vi "from string.vi"(8 "error in":errorcluster, 9 "data":string, 10 "version":string, 11 "J1939 configuration in":refnum<class "J1939 configuration.lvclass">) -> (0 "error out":errorcluster, 3 "J1939 configuration out":refnum<class "J1939 configuration.lvclass">)   [LabVIEW 2015, in "J1939 configuration.lvclass"]
doc: "Provides an interface for loading a module configuration from a file or other serialized data source. It is recommended that all children of this class store data in two sets--data required for its own initialization, and any data required for parent initialization--and that each implementation uses the <b>Call Parent Method</b> primitive to de-serialize parent information. As a result, it is expected that every module configuration class calls <b>component configuration.lvclass:From String.vi</b>."
uses:
  J1939 configuration.lvclass
  XNET Settings.ctl
  <vilib>/NI/Tag Bus Module Framework/channel/TBM channel.lvclass
  Line.ctl
  J1939 configuration.lvclass/J1939 configuration.ctl
  <vilib>/NI/Tag Bus Module Framework/module configuration/TBM module configuration.lvclass
  <vilib>/NI/Configuration Framework/serializable configuration/NISE_CEF_serializable configuration.lvclass
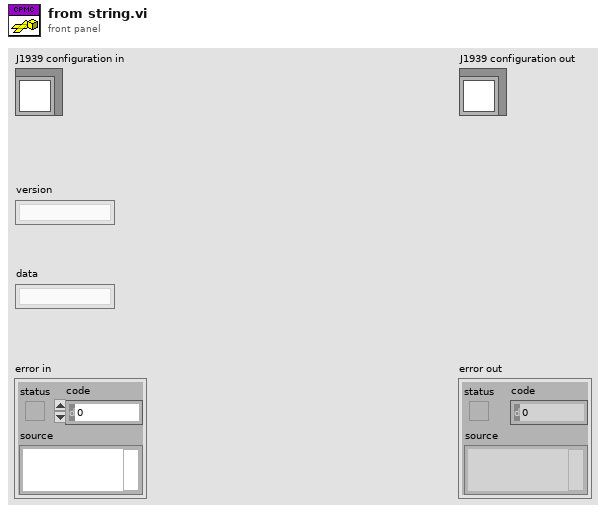
[diagram p1: front panel]
types:
  T1 = typedef "J1939 configuration.lvclass/XNET Settings.ctl" = cluster{"Select Interface":refnum<k21>, "Claim By Adress":bool, "Node Address":u8, "Node Name":u64}
  T2 = typedef "J1939 configuration.lvclass/Line.ctl" = cluster{"channel":refnum<class "TBM channel.lvclass">, "XNET Signal":refnum<k21>}
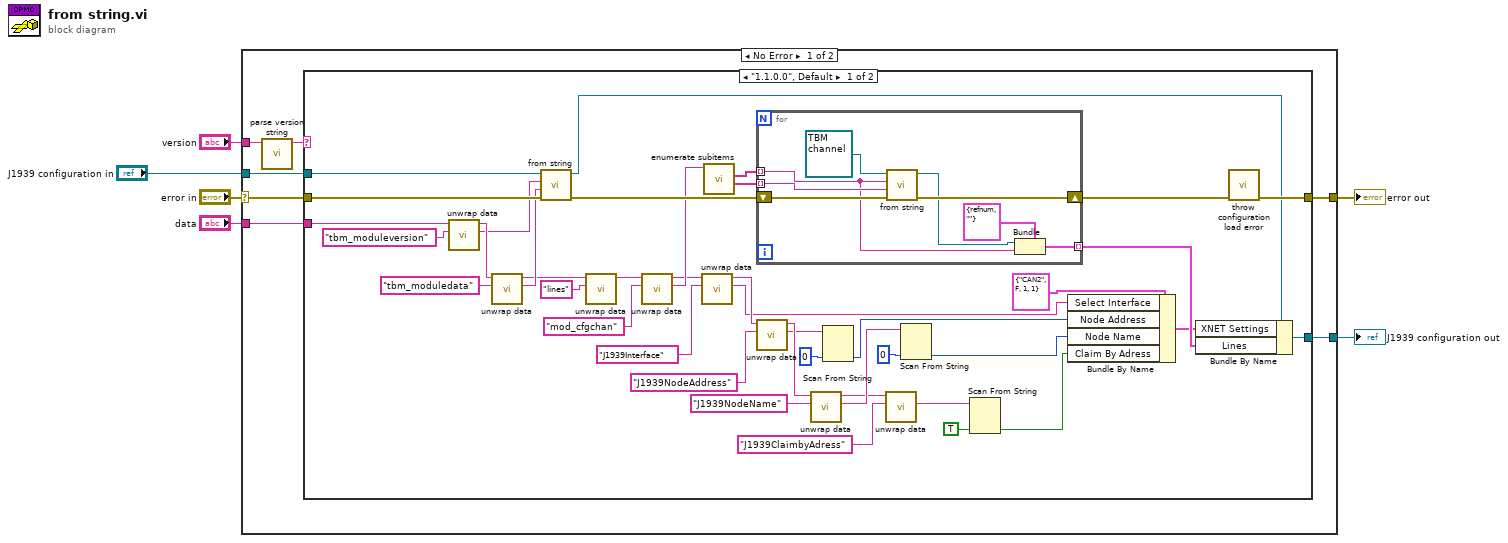
[diagram p0: block diagram]
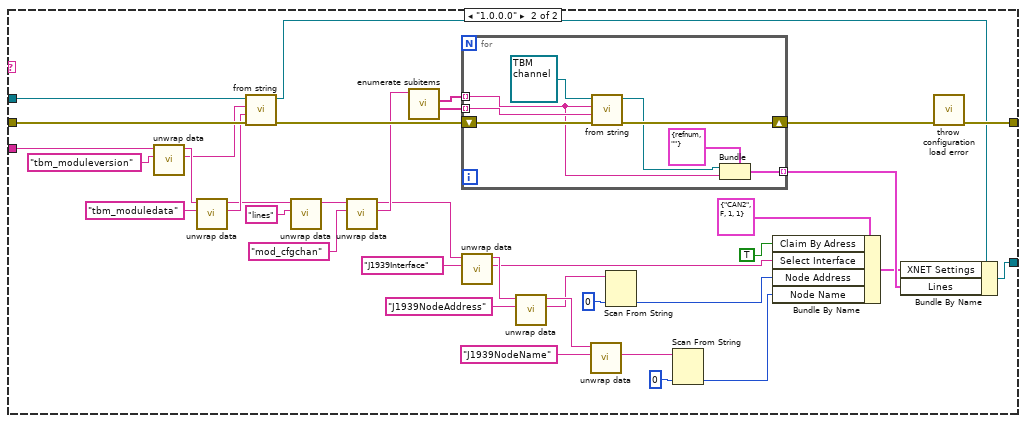
[diagram p2: hidden frame]
diagram:
  n1 = case shown="No Error" "error in" {
    selector: "error in" -> [w7 w109]
    tunnel: "data" -> [w13 _]
    tunnel: "J1939 configuration in" -> [w12 w108]
    tunnel: [w11 w108] -> w5
    tunnel: [w10 w109] -> w4
    tunnel: "version" -> [w9 _]
    frame No Error {
      n2 = call <vilib>:"parse version string.vi"("full version"=w9) -> ("major.minor version"=w8:string)  [unwired: 7 in, 3 out]
      n3 = case shown="\"1.1.0.0\", Default" w8 {
        tunnel: w13 -> [w51 w96]
        tunnel: w7 -> [w50 w95]
        tunnel: w12 -> [w54 w99]
        tunnel: [w42 w87] -> w11
        tunnel: [w53 w98] -> w10
        frame "1.1.0.0", Default {
          n4 = call <vilib>:"unwrap data.vi"("identifier"="tbm_moduleversion" ("additional identifier"), "data to unwrap"=w51) -> ("unwrapped data"=w46:string, "remaining string"=w52:string)  [unwired: 8 in]
          n5 = call <vilib>:"unwrap data.vi"("identifier"="tbm_moduledata" ("additional identifier"), "data to unwrap"=w52) -> ("unwrapped data"=w48:string, "remaining string"=w45:string)  [unwired: 8 in]
          n6 = call-parent "from string.vi"("error in"=w50, "data"=w48, "version"=w46, "module configuration in"=w54) -> ("error out"=w37:errorcluster, "module configuration out"=w43:refnum<class "J1939 configuration.lvclass">)  [unwired: 6 in]
          n7 = call <vilib>:"unwrap data.vi"("identifier"="lines" ("additional identifier"), "data to unwrap"=w45) -> ("remaining string"=w41:string)  [unwired: 8 in, 1 out]
          n8 = call <vilib>:"unwrap data.vi"("identifier"="mod_cfgchan", "data to unwrap"=w41) -> ("unwrapped data"=w36:string, "remaining string"=w33:string)  [unwired: 8 in]
          n9 = call <vilib>:"unwrap data.vi"("identifier"="J1939Interface", "data to unwrap"=w33) -> ("unwrapped data"=w26:string, "remaining string"=w30:string)  [unwired: 8 in]
          n10 = call <vilib>:"enumerate subitems.vi"("data to enumerate"=w36) -> ("associated data"=w38:string[], "discovered subitems"=w39:string[])  [unwired: 8 in, 1 out]
          n11 = for {
            shift-right: [w62] -> w34
            shift-left: w37 -> [w61]
            tunnel: w39 -> [w55] mode=indexing
            tunnel: w38 -> [w60] mode=indexing
            tunnel: [w56] -> w35 mode=indexing
            n12 = call-dynamic "from string.vi"("error in"=w61, "channel data"=w60, "identifier"=w55, "channel in"=refnum<class "TBM channel.lvclass"> refnum) -> ("error out"=w62:errorcluster, "channel out"=w57:refnum<class "TBM channel.lvclass">)  [unwired: 6 in]
            n13 = Bundle(cluster=T2 {"channel"=refnum, "XNET Signal"=""} ("Line"), "channel"=w57, "XNET Signal"=w55) -> (w56:T2)
          }
          n14 = call <vilib>:"unwrap data.vi"("identifier"="J1939NodeAddress", "data to unwrap"=w30) -> ("unwrapped data"=w23:string, "remaining string"=w29:string)  [unwired: 8 in]
          n15 = call <vilib>:"unwrap data.vi"("identifier"="J1939NodeName", "data to unwrap"=w29) -> ("unwrapped data"=w20:string, "remaining string"=w18:string)  [unwired: 8 in]
          n16 = Scan From String(input string=w23, default 1=u8 0 ("Node Address")) -> (output 1=w22:u8)  [unwired: 3 in, 3 out]
          n17 = call <vilib>:"unwrap data.vi"("identifier"="J1939ClaimbyAdress", "data to unwrap"=w18) -> ("unwrapped data"=w14:string)  [unwired: 8 in, 1 out]
          n18 = Scan From String(input string=w20, default 1=u8 0 ("Node Address")) -> (output 1=w21:u8)  [unwired: 3 in, 3 out]
          n19 = Scan From String(input string=w14, default 1=TRUE) -> (output 1=w15:bool)  [unwired: 3 in, 3 out]
          n20 = Bundle By Name(cluster=T1 {"Select Interface"="CAN2", "Claim By Adress"=FALSE, "Node Address"=1, "Node Name"=1} ("XNET Settings"), "Select Interface"=w26, "Node Address"=w22, "Node Name"=w21, "Claim By Adress"=w15) -> (w19:T1)
          n21 = Bundle By Name(cluster=w43, "XNET Settings"=w19, "Lines"=w35) -> (w42:refnum<class "J1939 configuration.lvclass">)
          n22 = call <vilib>:"throw configuration load error.vi"("error in"=w34) -> ("error out"=w53:errorcluster)  [unwired: 10 in]
        }
        frame "1.0.0.0" {
          n23 = call <vilib>:"unwrap data.vi"("identifier"="tbm_moduleversion" ("additional identifier"), "data to unwrap"=w96) -> ("unwrapped data"=w91:string, "remaining string"=w97:string)  [unwired: 8 in]
          n24 = call <vilib>:"unwrap data.vi"("identifier"="tbm_moduledata" ("additional identifier"), "data to unwrap"=w97) -> ("unwrapped data"=w93:string, "remaining string"=w90:string)  [unwired: 8 in]
          n25 = call-parent "from string.vi"("error in"=w95, "data"=w93, "version"=w91, "module configuration in"=w99) -> ("error out"=w82:errorcluster, "module configuration out"=w88:refnum<class "J1939 configuration.lvclass">)  [unwired: 6 in]
          n26 = call <vilib>:"unwrap data.vi"("identifier"="lines" ("additional identifier"), "data to unwrap"=w90) -> ("remaining string"=w86:string)  [unwired: 8 in, 1 out]
          n27 = call <vilib>:"unwrap data.vi"("identifier"="mod_cfgchan", "data to unwrap"=w86) -> ("unwrapped data"=w81:string, "remaining string"=w78:string)  [unwired: 8 in]
          n28 = call <vilib>:"enumerate subitems.vi"("data to enumerate"=w81) -> ("associated data"=w83:string[], "discovered subitems"=w84:string[])  [unwired: 8 in, 1 out]
          n29 = for {
            shift-right: [w107] -> w79
            shift-left: w82 -> [w106]
            tunnel: w84 -> [w100] mode=indexing
            tunnel: w83 -> [w105] mode=indexing
            tunnel: [w101] -> w80 mode=indexing
            n30 = call-dynamic "from string.vi"("error in"=w106, "channel data"=w105, "identifier"=w100, "channel in"=refnum<class "TBM channel.lvclass"> refnum) -> ("error out"=w107:errorcluster, "channel out"=w102:refnum<class "TBM channel.lvclass">)  [unwired: 6 in]
            n31 = Bundle(cluster=T2 {"channel"=refnum, "XNET Signal"=""} ("Line"), "channel"=w102, "XNET Signal"=w100) -> (w101:T2)
          }
          n32 = call <vilib>:"unwrap data.vi"("identifier"="J1939Interface", "data to unwrap"=w78) -> ("unwrapped data"=w71:string, "remaining string"=w75:string)  [unwired: 8 in]
          n33 = call <vilib>:"unwrap data.vi"("identifier"="J1939NodeAddress", "data to unwrap"=w75) -> ("unwrapped data"=w68:string, "remaining string"=w74:string)  [unwired: 8 in]
          n34 = call <vilib>:"unwrap data.vi"("identifier"="J1939NodeName", "data to unwrap"=w74) -> ("unwrapped data"=w65:string)  [unwired: 8 in, 1 out]
          n35 = Scan From String(input string=w68, default 1=u8 0 ("Node Address")) -> (output 1=w67:u8)  [unwired: 3 in, 3 out]
          n36 = Scan From String(input string=w65, default 1=u8 0 ("Node Address")) -> (output 1=w66:u8)  [unwired: 3 in, 3 out]
          n37 = Bundle By Name(cluster=T1 {"Select Interface"="CAN2", "Claim By Adress"=FALSE, "Node Address"=1, "Node Name"=1} ("XNET Settings"), "Claim By Adress"=TRUE, "Select Interface"=w71, "Node Address"=w67, "Node Name"=w66) -> (w64:T1)
          n38 = Bundle By Name(cluster=w88, "XNET Settings"=w64, "Lines"=w80) -> (w87:refnum<class "J1939 configuration.lvclass">)
          n39 = call <vilib>:"throw configuration load error.vi"("error in"=w79) -> ("error out"=w98:errorcluster)  [unwired: 10 in]
        }
      }
    }
    frame Error {
    }
  }
  "error out" <- w4
  "J1939 configuration out" <- w5
